vi "AlliGator VI Refnum Storage.vi"(6 "Get (F)/Set":bool, 8 "Error In":errorcluster, 10 "VI Refnum":refnum<vi>, 11 "VI Name":string) -> (0 "Error Out":errorcluster, 1 "Found?":bool, 2 "VI Refnum":refnum<vi>)   [LabVIEW 2021, in "AlliGator GUI.lvlib"]
uses:
  AlliGator GUI.lvlib
  <vilib>/Utility/error.llb/Error Cluster From Error Code.vi
  <vilib>/ErrorRing/Error Ring.xnode
panel:
  # "see the License on the block diagram (Ctrl+E or Window:Show Block Diagram)"
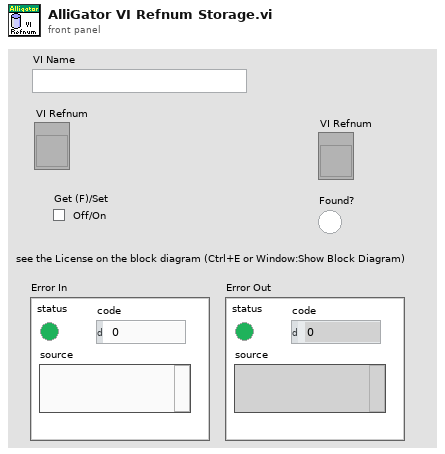
[diagram p1: front panel]
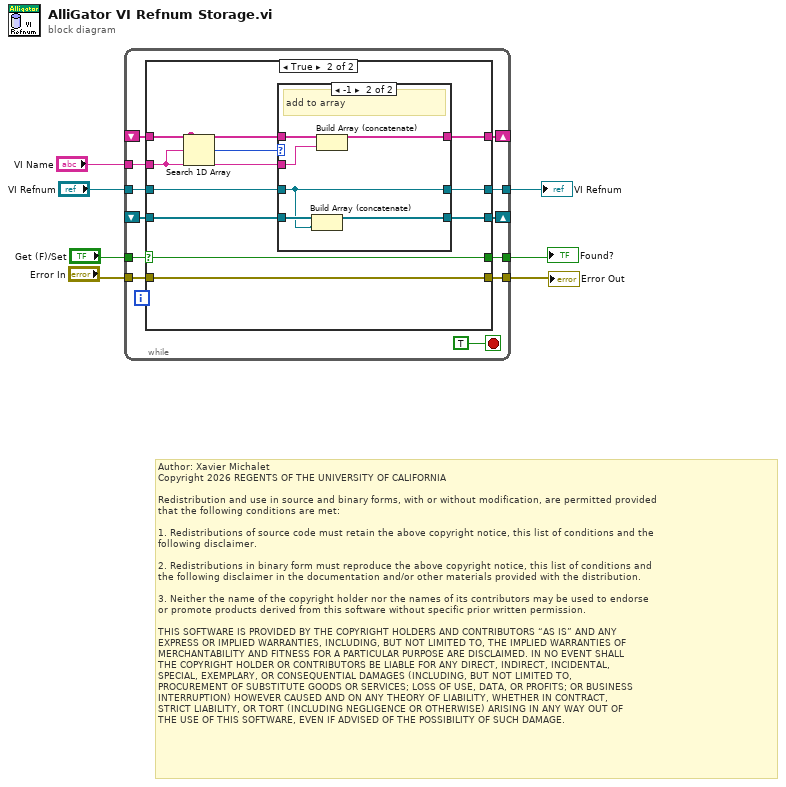
[diagram p0: block diagram]
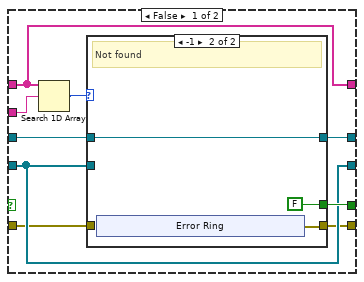
[diagram p2: hidden frame]
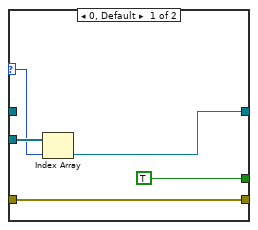
[diagram p3: hidden frame]
diagram:
  # "Author: Xavier Michalet\nCopyright 2026 REGENTS OF THE UNIVERSITY OF CALIFORNIA\n\nRedistribution and use in source and binary forms, with or without modification, are permitted provided\nthat the following conditions are met:\n\n1. Redistributions of source code must retain the above copyright notice, this list of conditions and the\nfollowing disclaimer.\n\n2. Redistributions in binary form must reproduce the above copyright notice, this list of conditions and\nthe following disclaimer in the documentation and/or other materials provided with the distribution.\n\n3. Neither the name of the copyright holder nor the names of its contributors may be used to endorse \nor promote products derived from this software without specific prior written permission.\n\nTHIS SOFTWARE IS PROVIDED BY THE COPYRIGHT HOLDERS AND CONTRIBUTORS “AS IS” AND ANY \nEXPRESS OR IMPLIED WARRANTIES, INCLUDING, BUT NOT LIMITED TO, THE IMPLIED WARRANTIES OF\nMERCHANTABILITY AND FITNESS FOR A PARTICULAR PURPOSE ARE DISCLAIMED. IN NO EVENT SHALL\nTHE COPYRIGHT HOLDER OR CONTRIBUTORS BE LIABLE FOR ANY DIRECT, INDIRECT, INCIDENTAL, \nSPECIAL, EXEMPLARY, OR CONSEQUENTIAL DAMAGES (INCLUDING, BUT NOT LIMITED TO, \nPROCUREMENT OF SUBSTITUTE GOODS OR SERVICES; LOSS OF USE, DATA, OR PROFITS; OR BUSINESS\nINTERRUPTION) HOWEVER CAUSED AND ON ANY THEORY OF LIABILITY, WHETHER IN CONTRACT, \nSTRICT LIABILITY, OR TORT (INCLUDING NEGLIGENCE OR OTHERWISE) ARISING IN ANY WAY OUT OF\nTHE USE OF THIS SOFTWARE, EVEN IF ADVISED OF THE POSSIBILITY OF SUCH DAMAGE."
  n1 = while {
    tunnel: "Get (F)/Set" -> [w18]
    shift-right: [w14] -> _
    shift-left: _ -> [w15]
    tunnel: "VI Refnum" -> [w17]
    tunnel: "VI Name" -> [w16]
    shift-right: [w12] -> _
    shift-left: _ -> [w13]
    tunnel: [w11] -> w4
    tunnel: [w10] -> w3
    tunnel: [w9] -> w2
    tunnel: "Error In" -> [w8]
    stop <- TRUE stop-if-true
    n2 = case shown="True" w18 {
      selector: w18 -> [_ w42]
      tunnel: w17 -> [w25 w45]
      tunnel: w16 -> [w28 w48]
      tunnel: w15 -> [w26 w49]
      tunnel: [w26 w47] -> w14
      tunnel: w13 -> [w22 w46]
      tunnel: [w22 w44] -> w12
      tunnel: [w24 w43] -> w11
      tunnel: [w23 w42] -> w10
      tunnel: [w21 w41] -> w9
      tunnel: w8 -> [w20 w41]
      frame False {
        n3 = Search 1D Array(1D array=w26, element=w28) -> (index of element=w27:i32)  [unwired: 1 in]
        n4 = case shown="-1" w27 {
          selector: w27 -> [w32 _]
          tunnel: w25 -> [_ w36]
          tunnel: [w31 w36] -> w24
          tunnel: [TRUE FALSE] -> w23
          tunnel: w22 -> [w33 _]
          tunnel: [w29 w34] -> w21
          tunnel: w20 -> [w29 _]
          frame 0, Default {
            n5 = Index Array(array=w33, index=w32) -> (element=w31:refnum<vi>)
          }
          frame -1 {
            # "Not found"
            n6 = xnode "Error Ring"() -> ("error out"=w34:errorcluster)
          }
        }
      }
      frame True {
        n7 = Search 1D Array(1D array=w49, element=w48) -> (index of element=w50:i32)  [unwired: 1 in]
        n8 = case shown="-1" w50 {
          tunnel: w49 -> [w53 w59]
          tunnel: w48 -> [_ w58]
          tunnel: [w53 w57] -> w47
          tunnel: w46 -> [w52 w56]
          tunnel: w45 -> [w51 w54]
          tunnel: [w52 w55] -> w44
          tunnel: [w51 w54] -> w43
          frame 0, Default {
            # "already exists: do nothing"
          }
          frame -1 {
            # "add to array"
            n9 = Build Array (concatenate)(w56, w54) -> (w55:refnum<vi>[])
            n10 = Build Array (concatenate)(w59, w58) -> (w57:string[])
          }
        }
      }
    }
  }
  "Error Out" <- w2
  "VI Refnum" <- w4
  "Found?" <- w3
